vi "CSE - Link Statement to Source Script.vi"(7 "get script source (T)":bool=TRUE, 8 "error in":errorcluster, 10 "Stm Index":i32, 11 "CSE RefNum":T1) -> (0 "error out":errorcluster, 1 "statement info":T3 {"stmType" items=["expression", "jump", "source ref", "jump stub", "source stub"]}, 2 "dup Stm Index":i32, 3 "dup CSE RefNum":T1, 4 "size":i32, 5 "script":string)   [LabVIEW 2021]
doc: "This VI returns information linking the specified statement in a parsed script to the script source. It also provides additional information reflecting the statement's attributes used for execution, debugging, and messaging. Refer to the VI help for more details.\n\n::: CalcExpress Toolkit :::\nCopyright (c) 2000-2026 Konstantin Shifershteyn. All rights reserved."
uses:
  CSE Instance RefNum.ctl
  cetypes.llb/CalcExpress Instance RefNum.ctl
  cersrc/celveng32.dll
panel:
  # "Source Info"
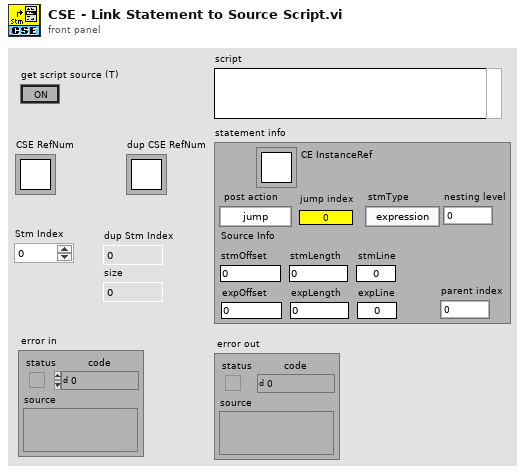
[diagram p1: front panel]
types:
  T1 = typedef "CSE Instance RefNum.ctl" = refnum<k1>
  T2 = typedef "CalcExpress Instance RefNum.ctl" = refnum<k1>
  T3 = cluster{"CE InstanceRef":T2, "post action":enum32{"jump", "jump if true", "jump if false", "stop"}, "jump index":i32, "stmType":i32, "nesting level":i32, "stmOffset":i32, "stmLength":i32, "stmLine ":i32, "expOffset":i32, "expLength":i32, "expLine":i32, "parent index":i32}
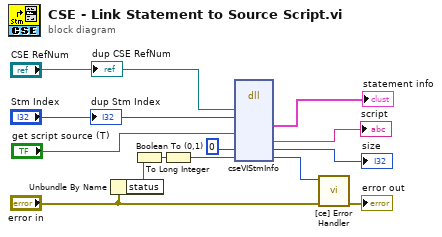
[diagram p0: block diagram]
diagram:
  n1 = Unbundle By Name("error in") -> ("status"=w9:bool)
  n2 = Boolean To (0,1)(Boolean=w9) -> (0, 1=w10:i16)
  n3 = To Long Integer(number=w10) -> (32bit integer=w6:i32)
  n4 = dll-call lib="C:/LV Projects/CalcExpress 40 LV2021/vi.lib/addons/CalcExpress/cersrc/celveng*.dll" fn="cseVIStmInfo"("iCESP"="CSE RefNum", "StmIndex"="Stm Index", "fGetScript"="get script source (T)", "arrSize"=0 ("errStat"), "errStat"=w6) -> ("statement info"=→"statement info":T3, "Script"=→"script":string, "arrSize"=→"size":i32, "errStat"=w5:i32)  [unwired: 9 in, 2 out]
  n5 = call "[ce] Error Handler.vi"("error in"="error in", "error code"=w5) -> ("error out"=→"error out":errorcluster)  [unwired: 8 in, 1 out]
  "dup Stm Index" <- "Stm Index"
  "dup CSE RefNum" <- "CSE RefNum"
